vi "DialogCloneMethod.vi"(0 "ClassWriterNative.lvclass":refnum<class "ClassWriterNative.lvclass">, 1 "VIItemRefIn":refnum<vi>, 5 "error in (no error)":errorcluster) -> (11 "NewVIDescriptionOut":string caption="New VI Description", 13 "OpenAfter":bool, 14 "ClassWriterGOOP300.lvclassOut":refnum<class "ClassWriterNative.lvclass">, 15 "VIItemRefOut":refnum<vi>, 16 "NewVIPath":path, 17 "Cancelled":bool, 18 "LibraryOwners":refnum<vi>[](array[refnum]), 19 "error out":errorcluster)   [LabVIEW 2020, in "ClassWriterNative.lvclass"]
uses:
  <resource>/Framework/Providers/Open_GDS/ClassProviders/Provider_LvNativeClass/ClassWriterNative_class/ClassWriterNative.lvclass
  8e0e01ac-982d-41f7-8aed-4e6b79215eef.vi
  8911d2c4-eda5-4945-b205-264938925bfc.vi
  63f0082b-caa7-4502-9d59-c3855e1c6e56.vi
  2d8d48ce-bc4c-4c8b-b501-0b6ffedba582.vi
  <vilib>/Utility/lvfile.llb/NI_FileType.lvlib
panel:
  in  "Help":bool
  out "ProductPicture":picture
  in  "_NewVIDescription":string caption="New VI Description"
  in  "_CreateOpenVI":bool
  in  "_OverwirteTragetVIs":bool
  out "_ViPathAlreadyExists":bool=TRUE caption="This VI already exists"
  out "_CloneViName":string caption="Original VI Name"
  in  "_ClassOwner":u16(ring) caption="New VI Owner" items=["<No owner selected>", "<Clone VI to Selected Classes>", "A.lvclass", "B.lvclass", "Base.lvclass", "C.lvclass", "C1.lvclass", "C2.lvclass", "D.lvclass", "E.lvclass", "F.lvclass", "F2.lvclass", "G1.lvclass", "G2.lvclass", "G3-B.lvclass", "G3.lvclass", "Hello.lvclass", "Sub.lvclass", "Test.lvclass", "X.lvclass"]
  in  "_ShowContextHelp":bool
  in  "_NewVIPath":path caption="New VI path"
  in  "_NewVIName":string caption="New VI name"
  in  "_Cancel":bool
  in  "_CloneVI":bool
  in  "_CloneMethodClasses":i32[](listbox) caption="Select which classes to clone the VI to"
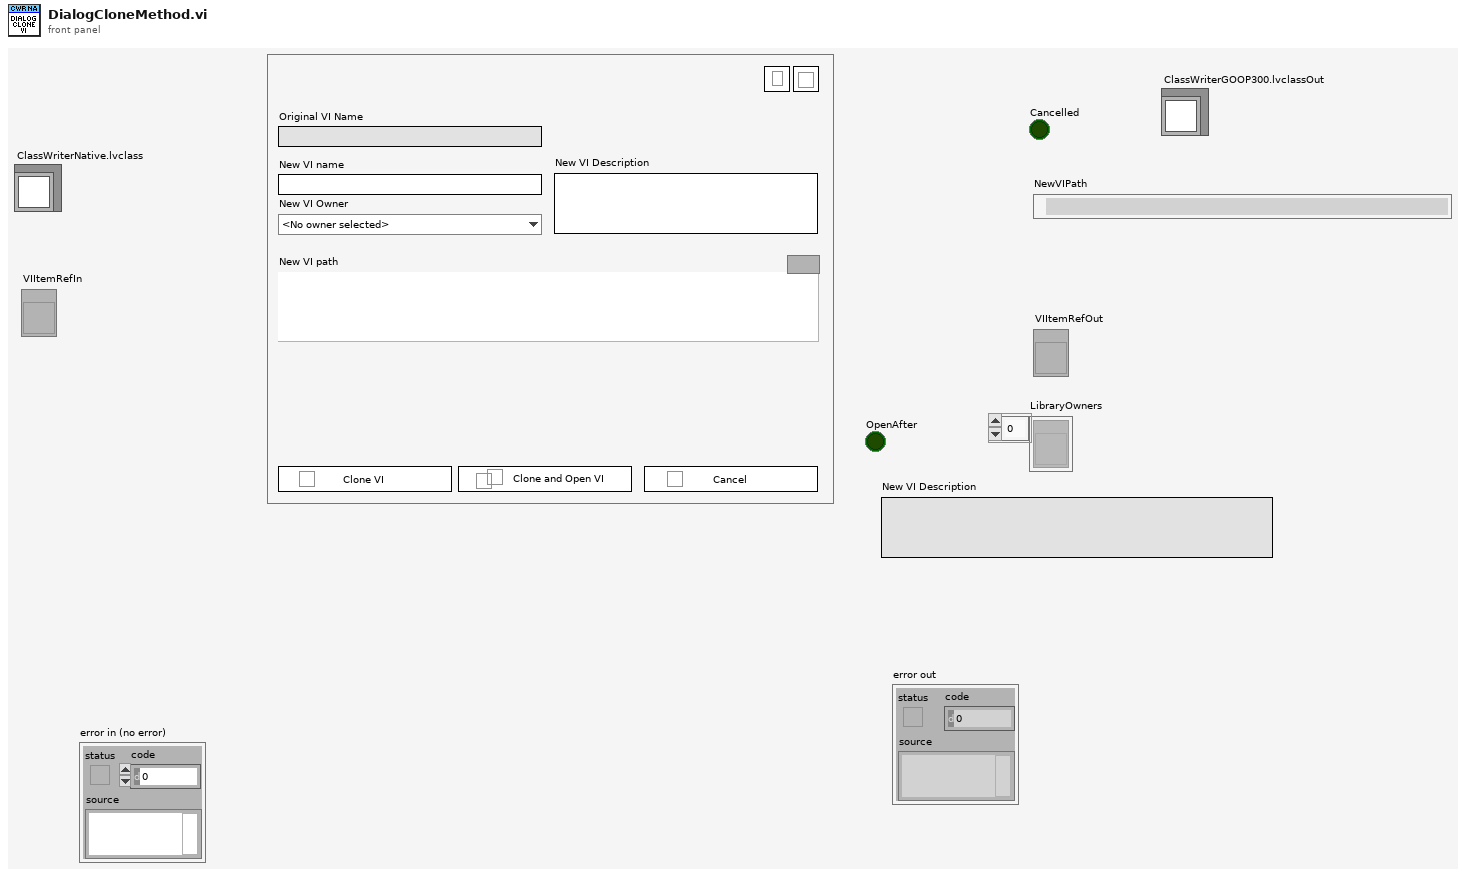
[diagram p1: front panel]
types:
  T1 = cluster{"Cancel":bool, "OrgVIPath":path, "VIName":string, "Libs":refnum<vi>[], "SiblingClasses":refnum<vi>[], "ProjectFolder":path, "ViRelFromParent":path, "OrgVIExt":string, "ManyClasses":bool, "OrgLibName":string, "AllClasses":refnum<vi>[], "OpenAfter":bool}
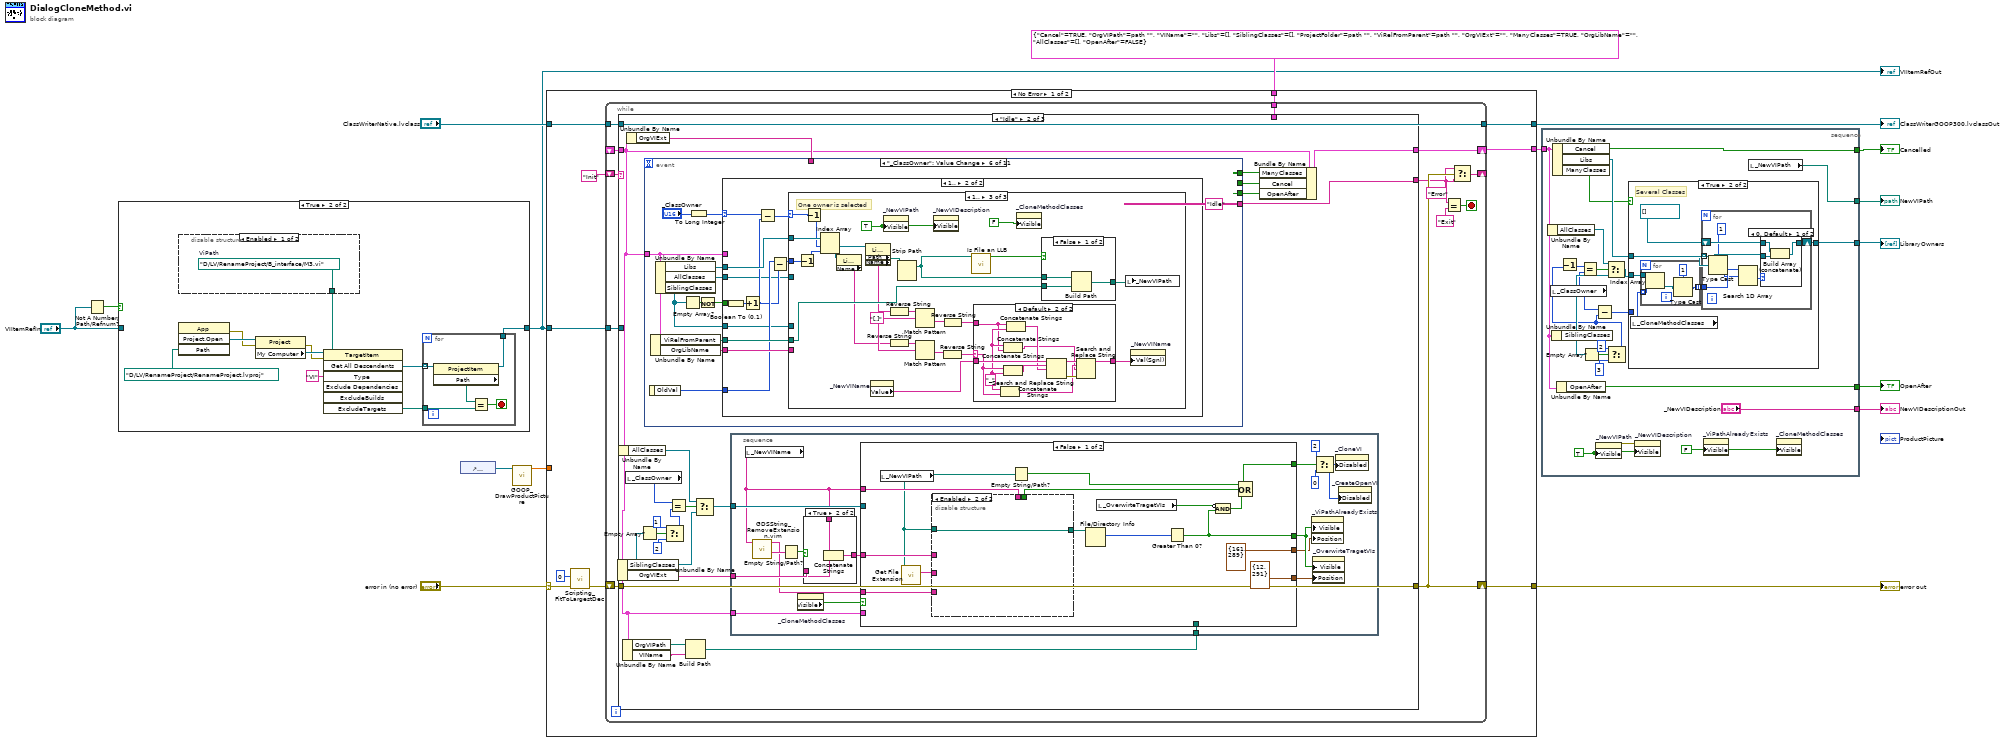
[diagram p0: block diagram]
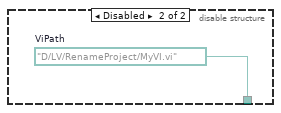
[diagram p3: hidden frame]
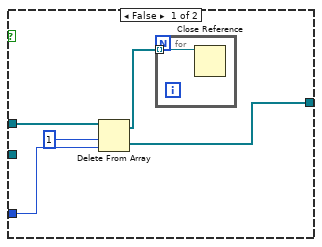
[diagram p4: hidden frame]
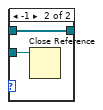
[diagram p5: hidden frame]
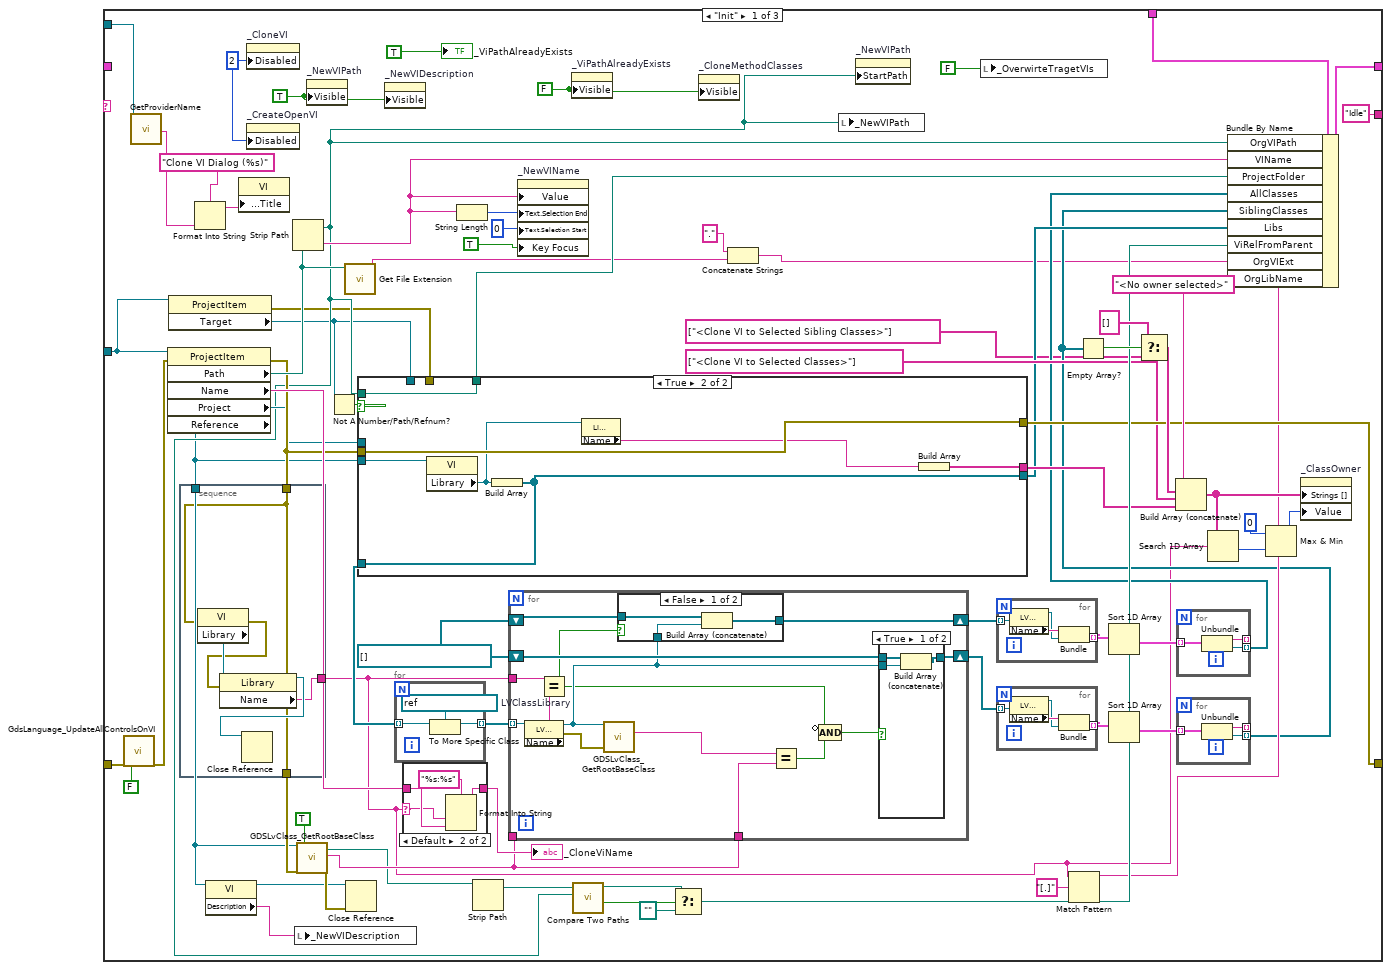
[diagram p6: hidden frame]
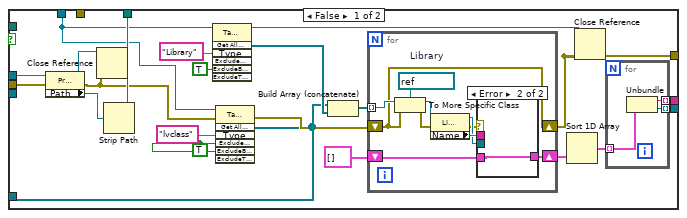
[diagram p7: hidden frame]
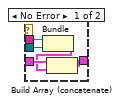
[diagram p8: hidden frame]
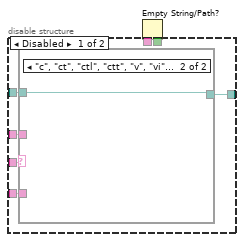
[diagram p13: hidden frame]
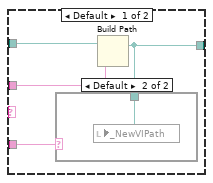
[diagram p14: hidden frame]
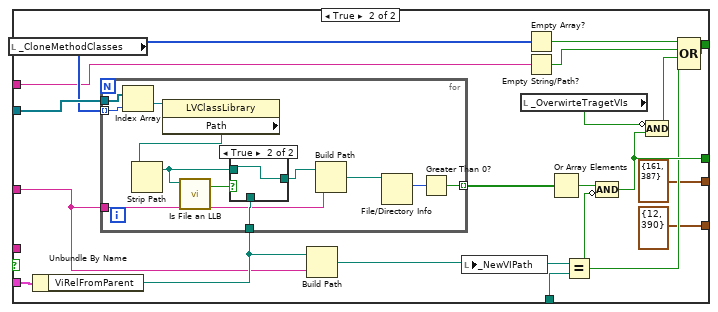
[diagram p16: hidden frame]
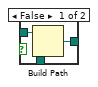
[diagram p17: hidden frame]
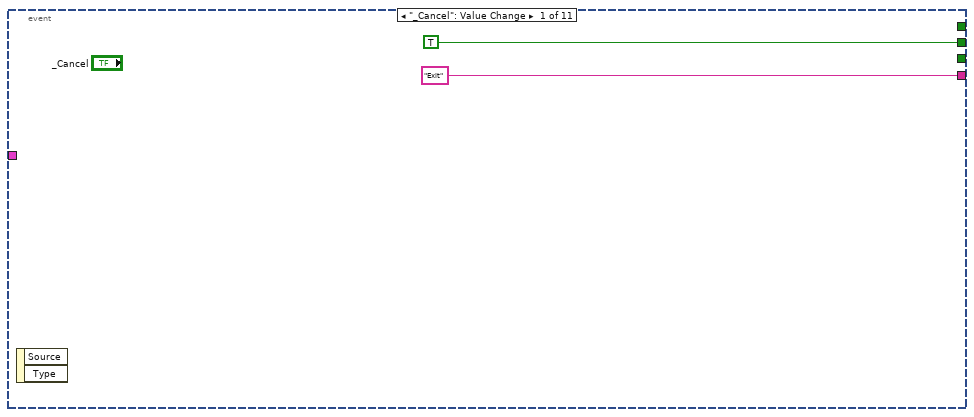
[diagram p18: hidden frame]
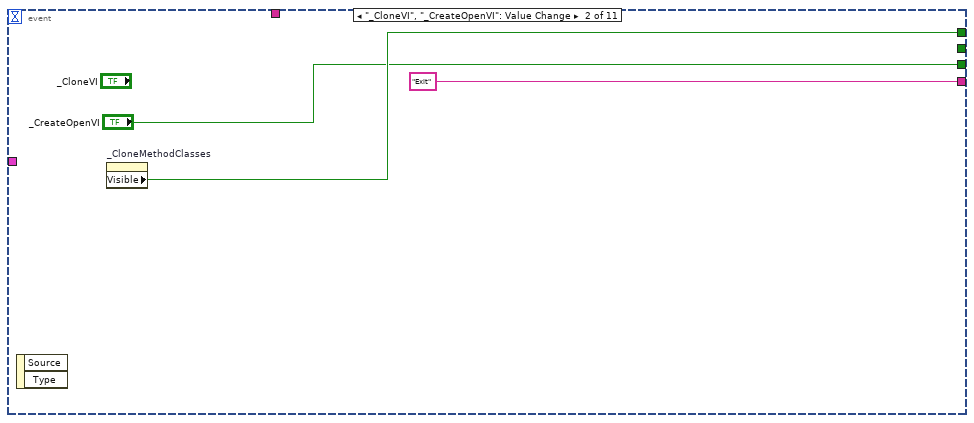
[diagram p19: hidden frame]
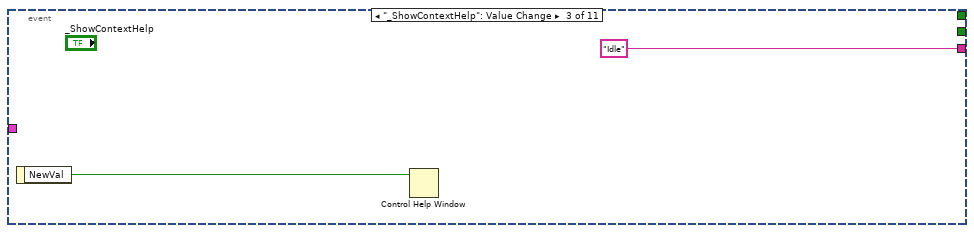
[diagram p20: hidden frame]
diagram:
  n1 = Not A Number/Path/Refnum?(number/path/refnum="VIItemRefIn") -> (NaN/Path/Refnum?=w3:bool)
  n2 = case shown="True" w3 {
    tunnel: "VIItemRefIn" -> [w17 _]
    tunnel: [w17 w18] -> w1
    frame False {
    }
    frame True {
      n3 = disable-structure shown="Enabled" {
        disable-tunnel: [w27 w28] -> w19
        frame Enabled {
          w27 = path "D:/LV/RenameProject/B_interface/M3.vi"  # ViPath
        }
        frame Disabled {
          w28 = path "D:/LV/RenameProject/MyVI.vi"  # ViPath
        }
      }
      n4 = invoke class="App" method="Project.Open"("Path"=path "D:/LV/RenameProject/RenameProject.lvproj") -> (error out=w21:errorcluster, "Project:Open"=w25:refnum<vi>)  [unwired: 3 in, 2 out]
      n5 = property class="Project"(reference=w25, error in=w21) -> (error out=w20:errorcluster, "My Computer"=w24:refnum<vi>)  [unwired: 1 out]
      n6 = invoke class="TargetItem" method="Get All Descendents"(reference=w24, error in=w20, "Type"="VI") -> ("All Descendents"=w22:refnum<vi>[])  [unwired: 4 in, 6 out]
      n7 = for {
        tunnel: w22 -> [w33] mode=indexing
        tunnel: w19 -> [w31]
        tunnel: [w29] -> w18
        stop <- w30 stop-if-true
        n8 = property class="ProjectItem"(reference=w33) -> (reference out=w29:refnum<vi>, "Path"=w32:path)  [unwired: 1 in, 1 out]
        n9 = Equal?(x=w32, y=w31) -> (x = y?=w30:bool)
      }
    }
  }
  "VIItemRefOut" <- w1
  n10 = control-ref of="ProductPicture"() -> (w5:refnum<vi>)
  n11 = call <resource>:"GOOP_DrawProductPicture.vi"("ProductPictureControl"=w5) -> ("Zoom Factor"=w4:sgl)  [unwired: 10 in]
  n12 = case shown="No Error" "error in (no error)" {
    selector: "error in (no error)" -> [w36 w493]
    tunnel: "ClassWriterNative.lvclass" -> [w41 w492]
    tunnel: [w43 w493] -> w11
    tunnel: [w42 w492] -> w14
    tunnel: T1 {"Cancel"=TRUE, "OrgVIPath"=path "", "VIName"="", "Libs"=[], "SiblingClasses"=[], "ProjectFolder"=path "", "ViRelFromParent"=path "", "OrgVIExt"="", "ManyClasses"=TRUE, "OrgLibName"="", "AllClasses"=[], "OpenAfter"=FALSE} ("output cluster") -> [w40 _]
    tunnel: w1 -> [w39 _]
    tunnel: [w38 _] -> w13
    tunnel: w4 -> [_ _]
    frame No Error {
      n13 = call <resource>:"Scripting_FitToLargestDec.vi"("error in (no error)"=w36, "border spacing (2 px)"=0) -> ("error out"=w35:errorcluster)  [unwired: 4 in, 1 out]
      n14 = while {
        shift-right: [w50] -> w43
        shift-left: w35 -> [w56]
        shift-right: [w49] -> _
        shift-left: "Init" -> [w53]
        shift-right: [w54] -> w38
        shift-left: _ -> [w55]
        tunnel: w41 -> [w46]
        tunnel: [w46] -> w42
        tunnel: w40 -> [w45]
        tunnel: w39 -> [w44]
        stop <- w51 stop-if-true
        n15 = case shown="\"Idle\"" w53 {
          tunnel: w55 -> [_ w231 w489]
          tunnel: [w128 w246 w488] -> w54
          tunnel: w56 -> [w120 w248 w490]
          tunnel: [w94 w248 w490] -> w50
          tunnel: w46 -> [w121 _ _]
          tunnel: ["Idle" w247 "Exit"] -> w48
          tunnel: w45 -> [w127 _ _]
          tunnel: w44 -> [w59 _ _]
          frame "Init" {
            w69 = TRUE ("Visible")
            w89 = refnum<vi>[] []
            w106 = FALSE ("Visible")
            w87 = u8 2 ("Disabled")
            n16 = call <resource>:"GdsLanguage_UpdateAllControlsOnVI.vi"("error in (no error)"=w120, "CreateLanguageFile(Use this to create a languageFile)"=FALSE) -> ("error out"=w119:errorcluster)  [unwired: 16 in, 1 out]
            n17 = call-dynamic "GetProviderName.vi"("ClassWriterNative in"=w121) -> ("TranslatedProviderName"=w66:string)  [unwired: 15 in, 3 out]
            n18 = property class="ProjectItem"(reference=w59, error in=w119) -> (error out=w72:errorcluster, "Path"=w99:path, "Name"=w96:string, "Project"=w63:refnum<vi>, "Reference"=w60:refnum<vi>)  [unwired: 1 out]
            n19 = property class="ProjectItem"(reference=w59) -> (error out=w57:errorcluster, "Target"=w58:refnum<vi>)  [unwired: 1 in, 1 out]
            n20 = stacked-sequence {
              tunnel: w60 -> [w183]
              tunnel: w72 -> [w179]
              tunnel: [w178] -> w70
              tunnel: [w179] -> w71
              frame #0 {
                n21 = property class="VI"(reference=w183, error in=w179) -> (error out=w181:errorcluster, "Library"=w182:refnum<vi>)  [unwired: 1 out]
                n22 = property class="Library"(reference=w182, error in=w181) -> (reference out=w180:refnum<vi>, "Name"=w178:string)  [unwired: 1 out]
                n23 = Close Reference(reference=w180) -> ()  [unwired: 1 in, 1 out]
              }
            }
            n24 = Format Into String(format string="Clone VI Dialog (%s)", w66) -> (resulting string=w123:string)  [unwired: 2 in, 1 out]
            n25 = property class="VI"(reference=w60) -> (reference out=w68:refnum<vi>, "Description"=w67:string)  [unwired: 1 in, 1 out]
            n26 = property class="VI"("Front Panel.Title"=w123) -> ()  [unwired: 2 in, 2 out]
            n27 = property on="_CloneVI" class="Bool"("Disabled"=w87) -> ()  [unwired: 2 in, 2 out]
            n28 = property on="_CreateOpenVI" class="Bool"("Disabled"=w87) -> ()  [unwired: 2 in, 2 out]
            n29 = Strip Path(path=w99) -> (stripped path=w61:path, name=w116:string)
            n30 = local write "_NewVIDescription"(w67) -> ()
            n31 = call <resource>:"GDSLvClass_GetRootBaseClass.vi"("ViRef/Path,LvClassRef/Path"=w60, "error in (no error)"=w71, "Don'tOpenReference"=TRUE) -> ("RootBaseClassPath"=w82:path, "ClassName"=w83:string, "error out"=w84:errorcluster)  [unwired: 10 in, 4 out]
            n32 = property on="_NewVIPath" class="Path"("Visible"=w69) -> ()  [unwired: 2 in, 2 out]
            n33 = Not A Number/Path/Refnum?(number/path/refnum=w58) -> (NaN/Path/Refnum?=w62:bool)
            n34 = call <vilib>:"Get File Extension.vi"("file"=w99) -> ("lowercase file extension"=w98:string)  [unwired: 6 in, 4 out]
            n35 = Close Reference(reference=w68, error in (no error)=w84) -> ()  [unwired: 1 out]
            n36 = case shown="True" w62 {
              tunnel: [w144 w174] -> w111
              tunnel: [w143 w177] -> w104
              tunnel: [w139 w176] -> w94
              tunnel: [w136 w171] -> w86
              tunnel: [w135 w174] -> w85
              tunnel: w72 -> [w134 w176]
              tunnel: w58 -> [w130 _]
              tunnel: w63 -> [w131 _]
              tunnel: w61 -> [_ w177]
              tunnel: w60 -> [_ w175]
              tunnel: w57 -> [_ _]
              frame False {
                w147 = TRUE ("ExcludeDependencies")
                w148 = TRUE ("ExcludeDependencies")
                n37 = property class="Project"(reference=w131, error in=w134) -> (reference out=w140:refnum<vi>, error out=w141:errorcluster, "Path"=w142:path)
                n38 = Close Reference(reference=w140, error in (no error)=w141) -> ()  [unwired: 1 out]
                n39 = Strip Path(path=w142) -> (stripped path=w143:path)  [unwired: 1 out]
                n40 = invoke class="TargetItem" method="Get All Descendents"(reference=w130, "Type"="Library", "Exclude Dependencies"=w148, "ExcludeBuilds"=w148) -> (reference out=w138:refnum<vi>, "All Descendents"=w146:refnum<vi>[])  [unwired: 3 in, 5 out]
                n41 = invoke class="TargetItem" method="Get All Descendents"(reference=w130, error in=w141, "Type"="lvclass", "Exclude Dependencies"=w147, "ExcludeBuilds"=w147) -> (error out=w150:errorcluster, "All Descendents"=w144:refnum<vi>[])  [unwired: 2 in, 5 out]
                n42 = Build Array (concatenate)(w144, w146) -> (w145:refnum<vi>[])
                n43 = for {
                  tunnel: w145 -> [w164] mode=indexing
                  shift-right: [w157] -> w139
                  shift-left: w150 -> [w157]
                  shift-right: [w155] -> w132
                  shift-left: cluster{"Name":string, refnum<vi>}[] [] -> [w156]
                  w162 = refnum<vi> refnum  # Library
                  n44 = To More Specific Class(target class=w162, reference=w164, error in=w157) -> (specific class reference=w163:refnum<vi>, error out=w161:errorcluster)
                  n45 = property class="Library"(reference=w163, error in=w161) -> (reference out=w159:refnum<vi>, error out=w158:errorcluster, "Name"=w160:string)
                  n46 = case shown="Error" w158 {
                    tunnel: w160 -> [w169 _]
                    tunnel: w159 -> [w168 _]
                    tunnel: w156 -> [w167 w170]
                    tunnel: [w165 w170] -> w155
                    frame No Error {
                      n47 = Bundle("Name"=w169, w168) -> (w166:cluster{"Name":string, refnum<vi>})  [unwired: 1 in]
                      n48 = Build Array (concatenate)(w167, w166) -> (w165:cluster{"Name":string, refnum<vi>}[])
                    }
                    frame Error {
                    }
                  }
                }
                n49 = Sort 1D Array(array=w132) -> (sorted array=w137:cluster{"Name":string, refnum<vi>}[])
                n50 = Close Reference(reference=w138, error in (no error)=w139) -> ()  [unwired: 1 out]
                n51 = for {
                  tunnel: w137 -> [w154] mode=indexing
                  tunnel: [w153] -> w136 mode=indexing
                  tunnel: [w152] -> w135 mode=indexing
                  n52 = Unbundle(w154) -> ("Name"=w153:string, w152:refnum<vi>)
                }
              }
              frame True {
                n53 = property class="VI"(reference=w175) -> ("Library"=w173:refnum<vi>)  [unwired: 1 in, 2 out]
                n54 = Build Array(w173) -> (w174:refnum<vi>[])
                n55 = property class="Library"(reference=w173) -> ("Name"=w172:string)  [unwired: 1 in, 2 out]
                n56 = Build Array(w172) -> (w171:string[])
              }
            }
            n57 = property on="_NewVIDescription" class="Str"("Visible"=w69) -> ()  [unwired: 2 in, 2 out]
            n58 = for {
              tunnel: w111 -> [w204] mode=indexing
              tunnel: [w203] -> w88 mode=indexing
              w205 = refnum<vi> refnum  # LVClassLibrary
              n59 = To More Specific Class(target class=w205, reference=w204) -> (specific class reference=w203:refnum<vi>)  [unwired: 1 in, 1 out]
            }
            n60 = case shown="Default" w70 {
              selector: w70 -> [_ w199]
              tunnel: w96 -> [w198 w201]
              tunnel: [w198 w200] -> w95
              frame "" {
              }
              frame Default {
                n61 = Format Into String(format string="%s:%s", w199, w201) -> (resulting string=w200:string)  [unwired: 2 in, 1 out]
              }
            }
            "_CloneViName" <- w95
            n62 = String Length(string=w116) -> (length=w124:i32)
            n63 = Strip Path(path=w82) -> (stripped path=w105:path)  [unwired: 1 out]
            n64 = for {
              tunnel: w88 -> [w219] mode=indexing
              tunnel: w83 -> [w210]
              shift-right: [w217] -> w74
              shift-left: w89 -> [w218]
              shift-right: [w214] -> w78
              shift-left: w89 -> [w215]
              tunnel: w83 -> [_]
              tunnel: w70 -> [w213]
              n65 = property class="LVClassLibrary"(reference=w219) -> (reference out=w212:refnum<vi>, error out=w211:errorcluster, "Name"=w216:string)  [unwired: 1 in]
              n66 = Equal?(x=w213, y=w216) -> (x = y?=w208:bool)
              n67 = call <resource>:"GDSLvClass_GetRootBaseClass.vi"("ViRef/Path,LvClassRef/Path"=w212, "error in (no error)"=w211) -> ("ClassName"=w209:string)  [unwired: 11 in, 6 out]
              n68 = case shown="False" w208 {
                tunnel: w215 -> [w222 w223]
                tunnel: w212 -> [w221 _]
                tunnel: [w220 w223] -> w214
                frame False {
                  n69 = Build Array (concatenate)(w222, w221) -> (w220:refnum<vi>[])
                }
                frame True {
                }
              }
              n70 = Equal?(x=w209, y=w210) -> (x = y?=w207:bool)
              n71 = Compound Arithmetic op=AND(invert w208, w207) -> (w206:bool)
              n72 = case shown="True" w206 {
                tunnel: w218 -> [w226 w227]
                tunnel: w212 -> [w225 _]
                tunnel: [w224 w227] -> w217
                frame True {
                  n73 = Build Array (concatenate)(w226, w225) -> (w224:refnum<vi>[])
                }
                frame False {
                }
              }
            }
            n74 = property on="_NewVIName" class="Str"("Value"=w116, "Text.Selection End"=w124, "Text.Selection Start"=u32 0 ("Text.Selection:Start"), "Key Focus"=TRUE) -> ()  [unwired: 2 in, 2 out]
            n75 = property on="_ViPathAlreadyExists" class="Bool (strict)"("Visible"=w106) -> ()  [unwired: 2 in, 2 out]
            n76 = call <vilib>:"Compare Two Paths.vi"("Path 2"=w61, "Path 1"=w105) -> ("Path 2 Relative to Path 1?"=w103:bool, "Relative Path from 1 to 2"=w102:path)  [unwired: 6 in, 2 out]
            n77 = Select(t=w102, s=w103, f=path "") -> (s? t:f=w100:path)
            n78 = property on="_CloneMethodClasses" class="LstBox (strict)"("Visible"=w106) -> ()  [unwired: 2 in, 2 out]
            n79 = Concatenate Strings("." ("string"), w98) -> (w64:string)
            n80 = local write "_NewVIPath"(w61) -> ()
            n81 = property on="_NewVIPath" class="Path"("StartPath"=w61) -> ()  [unwired: 2 in, 2 out]
            n82 = local write "_OverwirteTragetVIs"(FALSE ("Visible")) -> ()
            n83 = for {
              tunnel: w78 -> [w194] mode=indexing
              tunnel: [w195] -> w80 mode=indexing
              n84 = property class="LVClassLibrary"(reference=w194) -> (reference out=w196:refnum<vi>, "Name"=w197:string)  [unwired: 1 in, 1 out]
              n85 = Bundle("Name"=w197, w196) -> (w195:cluster{"Name":string, refnum<vi>})  [unwired: 1 in]
            }
            n86 = for {
              tunnel: w74 -> [w187] mode=indexing
              tunnel: [w188] -> w75 mode=indexing
              n87 = property class="LVClassLibrary"(reference=w187) -> (reference out=w189:refnum<vi>, "Name"=w190:string)  [unwired: 1 in, 1 out]
              n88 = Bundle("Name"=w190, w189) -> (w188:cluster{"Name":string, refnum<vi>})  [unwired: 1 in]
            }
            n89 = Match Pattern(string=w70, regular expression="[.]") -> (before substring=w92:string)  [unwired: 1 in, 3 out]
            n90 = Sort 1D Array(array=w80) -> (sorted array=w79:cluster{"Name":string, refnum<vi>}[])
            n91 = Sort 1D Array(array=w75) -> (sorted array=w76:cluster{"Name":string, refnum<vi>}[])
            n92 = for {
              tunnel: w79 -> [w193] mode=indexing
              tunnel: [w192] -> _ mode=indexing
              tunnel: [w191] -> w77 mode=indexing
              n93 = Unbundle(w193) -> ("Name"=w192:string, w191:refnum<vi>)
            }
            n94 = for {
              tunnel: w76 -> [w186] mode=indexing
              tunnel: [w185] -> _ mode=indexing
              tunnel: [w184] -> w73 mode=indexing
              n95 = Unbundle(w186) -> ("Name"=w185:string, w184:refnum<vi>)
            }
            n96 = Empty Array?(array=w73) -> (empty?=w109:bool)
            n97 = Select(t=string[] [], s=w109, f=string[] ["<Clone VI to Selected Sibling Classes>"]) -> (s? t:f=w108:string[])
            n98 = Build Array (concatenate)("<No owner selected>", w108, string[] ["<Clone VI to Selected Classes>"], w86) -> (w115:string[])
            n99 = Search 1D Array(1D array=w115, element=w70) -> (index of element=w114:i32)  [unwired: 1 in]
            n100 = Bundle By Name(cluster=w127, "OrgVIPath"=w61, "VIName"=w116, "ProjectFolder"=w104, "AllClasses"=w77, "SiblingClasses"=w73, "Libs"=w85, "ViRelFromParent"=w100, "OrgVIExt"=w64, "OrgLibName"=w92) -> (w128:T1)
            n101 = Max & Min(x=0 ("Text.Selection:Start"), y=w114) -> (max(x,y)=w112:i32)  [unwired: 1 out]
            n102 = property on="_ClassOwner" class="Ring (strict)"("Strings []"=w115, "Value"=w112) -> ()  [unwired: 2 in, 2 out]
            "_ViPathAlreadyExists" <- TRUE ("Visible")
          }
          frame "Idle" {
            n103 = Unbundle By Name(w231) -> ("SiblingClasses"=w237:refnum<vi>[], "OrgVIExt"=w243:string)
            n104 = Unbundle By Name(w231) -> ("AllClasses"=w240:refnum<vi>[])
            n105 = Unbundle By Name(w231) -> ("OrgVIPath"=w230:path, "VIName"=w229:string)
            n106 = local read "_ClassOwner"() -> (w235:u16)
            n107 = Unbundle By Name(w231) -> ("OrgVIExt"=w244:string)
            n108 = Empty Array?(array=w237) -> (empty?=w238:bool)
            n109 = event shown="[5] \"_ClassOwner\": Value Change" {
              selector: _ -> [_ _ _ _ _ _ _ _ _ _ _]
              dyn-events: _ -> [_ _ _ _ _ _ _ _ _ _ _]
              timeout: _ -> [_ _ _ _ _ _ _ _ _ _ _]
              tunnel: ["Exit" "Exit" "Idle" "Idle" "Idle" "Idle" "Idle" "Idle" "Idle" "Idle" "Exit"] -> w247
              tunnel: [TRUE _ _ _ _ _ _ _ _ _ w486] -> w245
              tunnel: w231 -> [_ _ _ _ w363 w396 _ _ _ _ _]
              tunnel: w244 -> [_ _ _ _ w365 _ _ _ _ _ _]
              tunnel: [_ w337 _ _ _ _ _ _ _ _ _] -> w242
              tunnel: [_ "_CreateOpenVI" _ _ _ _ _ _ _ _ _] -> w232
              event "_Cancel": Value Change {
                n110 = event-data() -> ()  [unwired: 1 in, 2 out]
              }
              event "_CloneVI", "_CreateOpenVI": Value Change {
                n111 = event-data() -> ()  [unwired: 1 in, 2 out]
                n112 = property on="_CloneMethodClasses" class="LstBox (strict)"() -> ("Visible"=w337:bool)  [unwired: 2 in, 2 out]
              }
              event "_ShowContextHelp": Value Change {
                n113 = event-data() -> ("NewVal"=w339:bool)  [unwired: 1 in]
                n114 = Control Help Window(1:w339) -> ()  [unwired: 1 in]
              }
              event "Help": Value Change {
                n115 = event-data() -> ()  [unwired: 1 in, 6 out]
                n116 = call <resource>:"GOOP_HelpMain.vi"() -> ()  [unwired: 12 in]
              }
              event "_NewVIName": Value Change {
                n117 = event-data() -> ()  [unwired: 1 in, 1 out]
                n118 = local read "_NewVIPath"() -> (w345:path)
                n119 = local read "_ClassOwner"() -> (w361:u16)
                n120 = Unbundle By Name(w363) -> ("OrgVIPath"=w362:path)  [unwired: 1 out]
                n121 = File/Directory Info(path=w345) -> (directory=w344:bool)  [unwired: 1 in, 6 out]
                n122 = call "GDSString_RemoveExtension.vim"("NameWithExtension"=w345) -> ("Extension"=w350:string)  [unwired: 9 in, 1 out]
                n123 = Strip Path(path=w345) -> (stripped path=w351:path)  [unwired: 1 out]
                n124 = Empty String/Path?(string/path=w350) -> (empty?=w343:bool)
                n125 = call <resource>:"GOOP300_RemoveUnwantedChars.vi"("StringIn"="_NewVIName") -> ("StringOut"=w352:string)  [unwired: 10 in]
                n126 = Or(x=w343, y=w344) -> (x .or. y?=w342:bool)
                n127 = call "GDSString_RemoveExtension.vim"("NameWithExtension"=w352) -> ("Extension"=w356:string, "NameWithoutExtension"=w353:string)  [unwired: 9 in]
                n128 = Select(t=w345, s=w342, f=w351) -> (s? t:f=w349:path)
                n129 = case shown="0" w361 {
                  tunnel: w362 -> [_ w368]
                  tunnel: [w367 w368] -> w348
                  tunnel: w349 -> [w367 _]
                  frame 0 {
                  }
                  frame Default {
                  }
                }
                n130 = Empty String/Path?(string/path=w353) -> (empty?=w355:bool)
                n131 = Empty String/Path?(string/path=w356) -> (empty?=w354:bool)
                n132 = call <vilib>:"Compare Two Paths.vi"("Path 2"=w349, "Path 1"=w348) -> ("Relative Path from 1 to 2"=w346:path)  [unwired: 6 in, 3 out]
                n133 = Build Path(base path=w348, name or relative path=w346) -> (appended path=w347:path)
                n134 = case shown="True" w355 {
                  tunnel: w347 -> [w372 w383]
                  tunnel: [w371 w384] -> w360
                  tunnel: w354 -> [w375 _]
                  tunnel: w353 -> [w374 _]
                  tunnel: w365 -> [w373 _]
                  tunnel: w352 -> [w370 _]
                  frame False {
                    n135 = case shown="False" w375 {
                      tunnel: w374 -> [_ w379]
                      tunnel: w373 -> [_ w378]
                      tunnel: [w376 w377] -> w369
                      tunnel: w370 -> [w376 _]
                      frame False {
                      }
                      frame True {
                        n136 = Concatenate Strings(w379, w378) -> (w377:string)
                      }
                    }
                    n137 = Build Path(base path=w372, name or relative path=w369) -> (appended path=w371:path)
                  }
                  frame True {
                    n138 = call "GDSString_RemoveExtension.vim"("NameWithExtension"=w383) -> ("Extension"=w385:string)  [unwired: 9 in, 1 out]
                    n139 = Strip Path(path=w383) -> (stripped path=w386:path)  [unwired: 1 out]
                    n140 = File/Directory Info(path=w383) -> (directory=w382:bool)  [unwired: 1 in, 6 out]
                    n141 = Empty String/Path?(string/path=w385) -> (empty?=w380:bool)
                    n142 = Or(x=w382, y=w380) -> (x .or. y?=w381:bool)
                    n143 = Select(t=w383, s=w381, f=w386) -> (s? t:f=w384:path)
                  }
                }
                n144 = Empty String/Path?(string/path=w360) -> (empty?=w358:bool)
                n145 = Not A Number/Path/Refnum?(number/path/refnum=w360) -> (NaN/Path/Refnum?=w359:bool)
                n146 = Or(x=w359, y=w358) -> (x .or. y?=w357:bool)
                n147 = case shown="False" w357 {
                  tunnel: w360 -> [w387 _]
                  frame False {
                    n148 = local write "_NewVIPath"(w387) -> ()
                  }
                  frame True {
                  }
                }
              }
              event "_ClassOwner": Value Change {
                n149 = event-data() -> ("OldVal"=w391:u16)  [unwired: 1 in]
                n150 = Unbundle By Name(w396) -> ("ViRelFromParent"=w395:path, "OrgLibName"=w392:string)
                n151 = Unbundle By Name(w396) -> ("Libs"=w397:refnum<vi>[], "AllClasses"=w388:refnum<vi>[], "SiblingClasses"=w389:refnum<vi>[])
                n152 = Empty Array?(array=w389) -> (empty?=w398:bool)
                n153 = To Long Integer(number="_ClassOwner") -> (32bit integer=w390:i32)
                n154 = Not(x=w398) -> (.not. x?=w393:bool)
                n155 = case shown="1.." w390 {
                  selector: w390 -> [_ w417]
                  tunnel: w396 -> [w405 _]
                  tunnel: w393 -> [_ w416]
                  tunnel: w397 -> [_ w414]
                  tunnel: w395 -> [_ w413]
                  tunnel: w392 -> [_ w412]
                  tunnel: w391 -> [_ w411]
                  tunnel: w389 -> [_ w407]
                  tunnel: w388 -> [_ w406]
                  frame 0, Default {
                    w400 = TRUE ("Visible")
                    # "No Owner is selected"
                    n156 = Unbundle By Name(w405) -> ("ProjectFolder"=w403:path)
                    n157 = property on="_NewVIName" class="Str"() -> ("Value"=w402:string)  [unwired: 2 in, 2 out]
                    n158 = property on="_CloneMethodClasses" class="LstBox (strict)"("Visible"=FALSE) -> ()  [unwired: 2 in, 2 out]
                    n159 = property on="_NewVIPath" class="Path"("Visible"=w400) -> (error out=w401:errorcluster)  [unwired: 2 in, 1 out]
                    n160 = local write "_NewVIPath"(w403) -> ()
                    n161 = property on="_NewVIName" class="Str"("Val(Sgnl)"=w402) -> ()  [unwired: 2 in, 2 out]
                    n162 = property on="_NewVIDescription" class="Str"(error in=w401, "Visible"=w400) -> ()  [unwired: 1 in, 2 out]
                  }
                  frame 1.. {
                    n163 = Boolean To (0,1)(Boolean=w416) -> (0, 1=w410:i16)
                    n164 = Increment(x=w410) -> (x+1=w408:i16)
                    n165 = Subtract(x=w417, y=w408) -> (x-y=w415:i32)
                    n166 = Subtract(x=w411, y=w408) -> (x-y=w409:u16)
                    n167 = case shown="1.." w415 {
                      selector: w415 -> [_ _ w460]
                      tunnel: w414 -> [_ _ w459]
                      tunnel: w413 -> [_ _ w452]
                      tunnel: w412 -> [_ _ _]
                      tunnel: w409 -> [_ _ w447]
                      tunnel: w407 -> [w421 _ _]
                      tunnel: w406 -> [_ w428 _]
                      frame -1, Default {
                        w418 = FALSE ("Visible")
                        # "Class Children selected"
                        n168 = for {
                          tunnel: [w426] -> w420 mode=indexing
                          tunnel: w421 -> [w425] mode=indexing
                          tunnel: [w424] -> w419 mode=indexing
                          i -> [w424]
                          n169 = property class="LVClassLibrary"(reference=w425) -> ("Name"=w426:string)  [unwired: 1 in, 2 out]
                        }
                        n170 = property on="_NewVIPath" class="Path"("Visible"=w418) -> ()  [unwired: 2 in, 2 out]
                        n171 = local write "_NewVIPath"(path "") -> ()
                        n172 = property on="_CloneMethodClasses" class="LstBox (strict)"("Item Names"=w420, "Value"=w419) -> ()  [unwired: 2 in, 2 out]
                        n173 = property on="_NewVIDescription" class="Str"("Visible"=w418) -> ()  [unwired: 2 in, 2 out]
                        n174 = property on="_CloneMethodClasses" class="LstBox (strict)"("Visible"=TRUE) -> ()  [unwired: 2 in, 2 out]
                      }
                      frame 0 {
                        w427 = FALSE ("Visible")
                        # "Any Class selected"
                        n175 = property on="_NewVIPath" class="Path"("Visible"=w427) -> ()  [unwired: 2 in, 2 out]
                        n176 = for {
                          tunnel: [w435] -> w430 mode=indexing
                          tunnel: w428 -> [w434] mode=indexing
                          tunnel: [w433] -> w429 mode=indexing
                          i -> [w433]
                          n177 = property class="LVClassLibrary"(reference=w434) -> ("Name"=w435:string)  [unwired: 1 in, 2 out]
                        }
                        n178 = local write "_NewVIPath"(path "") -> ()
                        n179 = property on="_NewVIDescription" class="Str"("Visible"=w427) -> ()  [unwired: 2 in, 2 out]
                        n180 = property on="_CloneMethodClasses" class="LstBox (strict)"("Item Names"=w430, "Value"=w429) -> ()  [unwired: 2 in, 2 out]
                        n181 = property on="_CloneMethodClasses" class="LstBox (strict)"("Visible"=TRUE) -> ()  [unwired: 2 in, 2 out]
                      }
                      frame 1.. {
                        w445 = "[.]" ("regular expression")
                        w443 = TRUE ("Visible")
                        # "One owner is selected"
                        n182 = Decrement(x=w447) -> (x-1=w448:u16)
                        n183 = Decrement(x=w460) -> (x-1=w458:i32)
                        n184 = Index Array(array=w459, index #1=w458, index #2=w448) -> (element #1=w457:refnum<vi>, element #2=w446:refnum<vi>)
                        n185 = property class="Library"(reference=w446) -> ("Name"=w437:string)  [unwired: 1 in, 2 out]
                        n186 = property class="Library"(reference=w457) -> ("Path"=w455:path, "Name"=w451:string)  [unwired: 1 in, 2 out]
                        n187 = property on="_NewVIName" class="Str"() -> ("Value"=w450:string)  [unwired: 2 in, 2 out]
                        n188 = property on="_NewVIPath" class="Path"("Visible"=w443) -> ()  [unwired: 2 in, 2 out]
                        n189 = Reverse String(1:w451) -> (0:w442:string)
                        n190 = Reverse String(1:w437) -> (0:w436:string)
                        n191 = Strip Path(path=w455) -> (stripped path=w453:path)  [unwired: 1 out]
                        n192 = Match Pattern(string=w442, regular expression=w445) -> (after substring=w441:string)  [unwired: 1 in, 3 out]
                        n193 = Match Pattern(string=w436, regular expression=w445) -> (after substring=w439:string)  [unwired: 1 in, 3 out]
                        n194 = property on="_NewVIDescription" class="Str"("Visible"=w443) -> ()  [unwired: 2 in, 2 out]
                        n195 = Reverse String(1:w439) -> (0:w438:string)
                        n196 = Reverse String(1:w441) -> (0:w440:string)
                        n197 = call <vilib>:"Is File an LLB.vi"("path"=w453) -> ("Is LLB?"=w454:bool)  [unwired: 9 in, 1 out]
                        n198 = case shown="Default" w438 {
                          selector: w438 -> [_ w471]
                          tunnel: w450 -> [w461 w472]
                          tunnel: w440 -> [_ w469]
                          tunnel: [w461 w462] -> w449
                          frame "" {
                          }
                          frame Default {
                            w470 = "_" ("string")
                            n199 = Concatenate Strings(w470, w471) -> (w464:string)
                            n200 = Concatenate Strings(w470, w469) -> (w463:string)
                            n201 = Concatenate Strings(w471, w470) -> (w468:string)
                            n202 = Concatenate Strings(w469, w470) -> (w467:string)
                            n203 = Search and Replace String(input string=w472, search string=w468, replace string=w467) -> (result string=w466:string, error out=w465:errorcluster)  [unwired: 5 in, 2 out]
                            n204 = Search and Replace String(input string=w466, search string=w464, replace string=w463, error in=w465) -> (result string=w462:string)  [unwired: 4 in, 3 out]
                          }
                        }
                        n205 = property on="_CloneMethodClasses" class="LstBox (strict)"("Visible"=FALSE) -> ()  [unwired: 2 in, 2 out]
                        n206 = case shown="False" w454 {
                          tunnel: w453 -> [w475 w476]
                          tunnel: w452 -> [w474 _]
                          tunnel: [w473 w476] -> w456
                          frame False {
                            n207 = Build Path(base path=w475, name or relative path=w474) -> (appended path=w473:path)
                          }
                          frame True {
                          }
                        }
                        n208 = local write "_NewVIPath"(w456) -> ()
                        n209 = property on="_NewVIName" class="Str"("Val(Sgnl)"=w449) -> ()  [unwired: 2 in, 2 out]
                      }
                    }
                  }
                }
              }
              event "_OverwirteTragetVIs": Value Change {
                n210 = event-data() -> ()  [unwired: 1 in, 3 out]
              }
              event "_CloneMethodClasses": Value Change {
                n211 = event-data() -> ()  [unwired: 1 in, 1 out]
              }
              event "_CloneMethodClasses": Shortcut Menu Selection (User) {
                n212 = event-data() -> ()  [unwired: 1 in, 1 out]
                n213 = property on="_CloneMethodClasses" class="LstBox (strict)"() -> ("Item Names"=w479:string[])  [unwired: 2 in, 2 out]
                n214 = for {
                  tunnel: [w482] -> w481 mode=indexing
                  tunnel: w479 -> [_] mode=indexing
                  i -> [w482]
                }
                n215 = local write "_CloneMethodClasses"(w481) -> ()
              }
              event "_NewVIPath": Value Change {
                n216 = event-data() -> ()  [unwired: 1 in, 4 out]
                n217 = property on="_NewVIName" class="Str"() -> ("Value"=w483:string)  [unwired: 2 in, 2 out]
                n218 = property on="_NewVIName" class="Str"("Val(Sgnl)"=w483) -> ()  [unwired: 2 in, 2 out]
              }
              event Panel Close? {
                w486 = TRUE ("Discard?")
                n219 = event-data() -> ()  [unwired: 1 in, 4 out]
                n220 = event-data("Discard?"=w486) -> ()  [unwired: 1 in, 1 out]
              }
            }
            n221 = Select(t=u16 1 ("x"), s=w238, f=u16 2 ("x")) -> (s? t:f=w234:u16)
            n222 = Equal?(x=w235, y=w234) -> (x = y?=w236:bool)
            n223 = Build Path(base path=w230, name or relative path=w229) -> (appended path=w228:path)
            n224 = Select(t=w240, s=w236, f=w237) -> (s? t:f=w241:refnum<vi>[])
            n225 = stacked-sequence {
              tunnel: w243 -> [w262]
              tunnel: w241 -> [w260]
              tunnel: w231 -> [w259]
              tunnel: w228 -> [w255]
              frame #0 {
                n226 = local read "_NewVIName"() -> (w250:string)
                n227 = call "GDSString_RemoveExtension.vim"("NameWithExtension"=w250) -> ("Extension"=w252:string, "NameWithoutExtension"=w249:string)  [unwired: 9 in]
                n228 = Empty String/Path?(string/path=w252) -> (empty?=w251:bool)
                n229 = property on="_CloneMethodClasses" class="LstBox (strict)"() -> ("Visible"=w261:bool)  [unwired: 2 in, 2 out]
                n230 = case shown="True" w251 {
                  tunnel: [w266 w269] -> w263
                  tunnel: w250 -> [w266 w268]
                  tunnel: w262 -> [_ w267]
                  frame False {
                  }
                  frame True {
                    n231 = Concatenate Strings(w268, w267) -> (w269:string)
                  }
                }
                n232 = case shown="False" w261 {
                  tunnel: [w284 w313] -> w258
                  tunnel: w263 -> [w283 w311]
                  tunnel: w250 -> [w278 w308]
                  tunnel: [w275 w302] -> w257
                  tunnel: w260 -> [_ w317]
                  tunnel: w259 -> [_ w316]
                  tunnel: w255 -> [_ w304]
                  tunnel: [cluster{"Left":i32, "Top":i32} {"Left"=12, "Top"=291} ("Position") cluster{"Left":i32, "Top":i32} {"Left"=12, "Top"=390} ("Position")] -> w254
                  tunnel: [cluster{"Left":i32, "Top":i32} {"Left"=161, "Top"=289} ("Position") cluster{"Left":i32, "Top":i32} {"Left"=161, "Top"=387} ("Position")] -> w253
                  tunnel: w249 -> [w270 _]
                  frame False {
                    n233 = local read "_NewVIPath"() -> (w277:path)
                    n234 = call <vilib>:"Get File Extension.vi"("file"=w277) -> ("lowercase file extension"=w276:string)  [unwired: 6 in, 4 out]
                    n235 = disable-structure shown="Enabled" {
                      disable-tunnel: w283 -> [w291 _]
                      disable-tunnel: [w290 w298] -> w282
                      disable-tunnel: [w289 _] -> w280
                      disable-tunnel: w278 -> [w288 _]
                      disable-tunnel: w277 -> [w287 w298]
                      disable-tunnel: w276 -> [w286 _]
                      disable-tunnel: w270 -> [w285 _]
                      frame Disabled {
                        n236 = case shown="\"c\", \"ct\", \"ctl\", \"ctt\", \"v\", \"vi\", \"vim\", \"vit\"" w286 {
                          tunnel: w291 -> [w295 _]
                          tunnel: [w293 w297] -> w290
                          tunnel: w287 -> [w294 w297]
                          tunnel: w285 -> [w292 _]
                          frame Default {
                            n237 = Build Path(base path=w294, name or relative path=w295) -> (appended path=w293:path)
                            n238 = case shown="Default" w292 {
                              tunnel: w293 -> [_ w296]
                              frame "" {
                              }
                              frame Default {
                                n239 = local write "_NewVIPath"(w296) -> ()
                              }
                            }
                          }
                          frame "c", "ct", "ctl", "ctt", "v", "vi", "vim", "vit" {
                          }
                        }
                        n240 = Empty String/Path?(string/path=w288) -> (empty?=w289:bool)
                      }
                      frame Enabled {
                      }
                    }
                    n241 = Empty String/Path?(string/path=w277) -> (empty?=w279:bool)
                    n242 = File/Directory Info(path=w282) -> (size=w281:i64)  [unwired: 1 in, 6 out]
                    n243 = local read "_OverwirteTragetVIs"() -> (w273:bool)
                    n244 = Greater Than 0?(x=w281) -> (x > 0?=w275:bool)
                    n245 = Compound Arithmetic op=AND(invert w273, w275) -> (w274:bool)
                    n246 = Compound Arithmetic op=OR(w279, w280, w274) -> (w284:bool)
                  }
                  frame True {
                    n247 = local read "_CloneMethodClasses"() -> (w310:i32[])
                    n248 = Unbundle By Name(w316) -> ("ViRelFromParent"=w312:path)
                    n249 = for {
                      tunnel: w317 -> [w329]
                      tunnel: w310 -> [w328] mode=indexing
                      tunnel: w312 -> [w325]
                      tunnel: w311 -> [w323]
                      tunnel: [w320] -> w315 mode=indexing
                      n250 = Index Array(array=w329, index=w328) -> (element=w327:refnum<vi>)
                      n251 = property class="LVClassLibrary"(reference=w327) -> ("Path"=w326:path)  [unwired: 1 in, 2 out]
                      n252 = Strip Path(path=w326) -> (stripped path=w319:path)  [unwired: 1 out]
                      n253 = call <vilib>:"Is File an LLB.vi"("path"=w319) -> ("Is LLB?"=w318:bool)  [unwired: 9 in, 1 out]
                      n254 = case shown="True" w318 {
                        tunnel: w325 -> [w332 _]
                        tunnel: [w331 w333] -> w324
                        tunnel: w319 -> [w330 w333]
                        frame False {
                          n255 = Build Path(base path=w330, name or relative path=w332) -> (appended path=w331:path)
                        }
                        frame True {
                        }
                      }
                      n256 = Build Path(base path=w324, name or relative path=w323) -> (appended path=w321:path)
                      n257 = File/Directory Info(path=w321) -> (size=w322:i64)  [unwired: 1 in, 6 out]
                      n258 = Greater Than 0?(x=w322) -> (x > 0?=w320:bool)
                    }
                    n259 = Build Path(base path=w312, name or relative path=w311) -> (appended path=w305:path)
                    n260 = local write "_NewVIPath"(w305) -> ()
                    n261 = local read "_OverwirteTragetVIs"() -> (w307:bool)
                    n262 = Empty Array?(array=w310) -> (empty?=w309:bool)
                    n263 = Empty String/Path?(string/path=w308) -> (empty?=w314:bool)
                    n264 = Or Array Elements(Boolean array=w315) -> (logical OR=w303:bool)
                    n265 = Equal?(x=w305, y=w304) -> (x = y?=w301:bool)
                    n266 = Compound Arithmetic op=AND(w303, invert w301) -> (w302:bool)
                    n267 = Compound Arithmetic op=AND(invert w307, w302) -> (w306:bool)
                    n268 = Compound Arithmetic op=OR(w309, w314, w306, w301) -> (w313:bool)
                  }
                }
                n269 = property on="_ViPathAlreadyExists" class="Bool (strict)"("Visible"=w257, "Position"=w253) -> ()  [unwired: 2 in, 2 out]
                n270 = property on="_OverwirteTragetVIs" class="Bool (strict)"("Visible"=w257, "Position"=w254) -> ()  [unwired: 2 in, 2 out]
                n271 = Select(t=u8 2, s=w258, f=u8 0 ("Disabled")) -> (s? t:f=w256:u8)
                n272 = property on="_CloneVI" class="Bool"("Disabled"=w256) -> ()  [unwired: 2 in, 2 out]
                n273 = property on="_CreateOpenVI" class="Bool"("Disabled"=w256) -> ()  [unwired: 2 in, 2 out]
              }
            }
            n274 = Bundle By Name(cluster=w231, "ManyClasses"=w242, "Cancel"=w245, "OpenAfter"=w232) -> (w246:T1)
          }
          frame "Error", Default {
            n275 = Bundle By Name(cluster=w489, "Cancel"=TRUE) -> (w488:T1)
          }
        }
        n276 = Equal?(x=w48, y="Exit") -> (x = y?=w51:bool)
        n277 = Select(t="Error", s=w50, f=w48) -> (s? t:f=w49:string)
      }
    }
    frame Error {
    }
  }
  "ClassWriterGOOP300.lvclassOut" <- w14
  "error out" <- w11
  n278 = stacked-sequence {
    tunnel: w13 -> [w498]
    tunnel: [w515] -> w12
    tunnel: [w512] -> w9
    tunnel: [w507] -> w8
    tunnel: [w497] -> w7
    tunnel: ["_NewVIDescription"] -> w6
    frame #0 {
      w495 = TRUE ("Visible")
      w514 = FALSE ("Visible")
      n279 = Unbundle By Name(w498) -> ("AllClasses"=w503:refnum<vi>[])
      n280 = local read "_ClassOwner"() -> (w502:u16)
      n281 = Unbundle By Name(w498) -> ("SiblingClasses"=w505:refnum<vi>[])
      n282 = Unbundle By Name(w498) -> ("Cancel"=w515:bool, "Libs"=w513:refnum<vi>[], "ManyClasses"=w506:bool)
      n283 = Unbundle By Name(w498) -> ("OpenAfter"=w497:bool)
      n284 = Empty Array?(array=w505) -> (empty?=w511:bool)
      n285 = property on="_NewVIPath" class="Path"("Visible"=w495) -> (error out=w496:errorcluster)  [unwired: 2 in, 1 out]
      n286 = Select(t=u16 2 ("x"), s=w511, f=u16 3 ("x")) -> (s? t:f=w499:u16)
      n287 = Decrement(x=w499) -> (x-1=w500:u16)
      n288 = Equal?(x=w500, y=w502) -> (x = y?=w501:bool)
      n289 = Subtract(x=w502, y=w499) -> (x-y=w508:u16)
      n290 = Select(t=w503, s=w501, f=w505) -> (s? t:f=w504:refnum<vi>[])
      n291 = case shown="True" w506 {
        tunnel: w513 -> [w520 w527]
        tunnel: [w517 w525] -> w512
        tunnel: w508 -> [w519 _]
        tunnel: w504 -> [_ w524]
        frame False {
          n292 = Delete From Array(array=w520, length=1, index=w519) -> (deleted portion=w517:refnum<vi>[], array with subset deleted=w516:refnum<vi>[])
          n293 = for {
            tunnel: w516 -> [w521] mode=indexing
            n294 = Close Reference(reference=w521) -> ()  [unwired: 1 in, 1 out]
          }
        }
        frame True {
          # "Several Classes"
          n295 = local read "_CloneMethodClasses"() -> (w523:i32[])
          n296 = for {
            tunnel: w524 -> [w532]
            tunnel: w523 -> [w531] mode=indexing
            tunnel: [w529] -> w522 mode=indexing
            n297 = Index Array(array=w532, index=w531) -> (element=w530:refnum<vi>)
            n298 = Type Cast(type=u32 1 ("x"), x=w530) -> (*(type *) &x=w529:u32)
          }
          n299 = for {
            tunnel: w527 -> [w535] mode=indexing
            shift-right: [w538] -> w525
            shift-left: refnum<vi>[] [] -> [w539]
            tunnel: w522 -> [w536]
            n300 = Type Cast(type=u32 1 ("x"), x=w535) -> (*(type *) &x=w533:u32)
            n301 = Search 1D Array(1D array=w536, element=w533) -> (index of element=w537:i32)  [unwired: 1 in]
            n302 = case shown="0, Default" w537 {
              tunnel: w535 -> [w542 w543]
              tunnel: w539 -> [w541 w544]
              tunnel: [w540 w544] -> w538
              frame 0, Default {
                n303 = Build Array (concatenate)(w541, w542) -> (w540:refnum<vi>[])
              }
              frame -1 {
                n304 = Close Reference(reference=w543) -> ()  [unwired: 1 in, 1 out]
              }
            }
          }
        }
      }
      n305 = property on="_NewVIDescription" class="Str"(error in=w496, "Visible"=w495) -> ()  [unwired: 1 in, 2 out]
      n306 = property on="_ViPathAlreadyExists" class="Bool (strict)"("Visible"=w514) -> ()  [unwired: 2 in, 2 out]
      n307 = local read "_NewVIPath"() -> (w507:path)
      n308 = property on="_CloneMethodClasses" class="LstBox (strict)"("Visible"=w514) -> ()  [unwired: 2 in, 2 out]
    }
  }
  "Cancelled" <- w12
  "NewVIPath" <- w8
  "LibraryOwners" <- w9
  "OpenAfter" <- w7
  "NewVIDescriptionOut" <- w6
